vi "VIH HelpGen - Image - Find Ctrl Area in Conpane Picture - Preparation.vi"(9 "Ctrl Attributes":T2[](array[typedef]), 10 "Term Names":string[](array[string]), 11 "Ctrl Labels":string[](array[string])) -> (0 "Max Column - Indicators":i32, 1 "Max Column - Controls":i32, 3 "Params":T1(array[cluster]) {"Name image" format="%.0x"})   [LabVIEW 2014]
doc: "::: VI Helpeks :::\nCopyright (c) 2000-2026 Konstantin Shifershteyn. All rights reserved."
uses:
  VIH HelpGen Typedef - Control Terminal Attributes Cluster.ctl
panel:
  # "VI Helpeks\nCopyright (c) 2012-2026 Konstantin Shifershteyn"
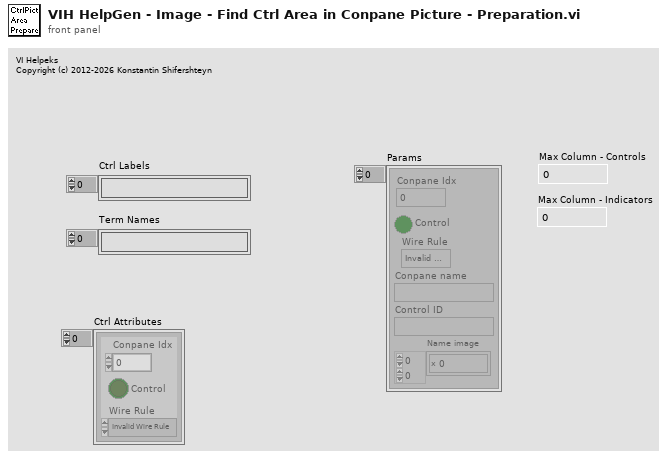
[diagram p1: front panel]
types:
  T1 = cluster{"Conpane Idx":i32, "Control":bool, "Wire Rule":enum16{"Invalid Wire Rule", "Required", "Recommended", "Optional", "Dynamic Dispatch"}, "Conpane name":string, "Control ID":string, "Name image":u32[][]}[]
  T2 = typedef "VIH HelpGen Typedef - Control Terminal Attributes Cluster.ctl" = cluster{"Conpane Idx":i32, "Control":bool, "Wire Rule":enum16{"Invalid Wire Rule", "Required", "Recommended", "Optional", "Dynamic Dispatch"}}
  T3 = cluster{i32, "Conpane name out":string, "Control ID":string, i32}
  T4 = cluster{i32, "Conpane name out":string, "Control ID":string, i32}[]
  T5 = enum16{"Invalid Wire Rule", "Required", "Recommended", "Optional", "Dynamic Dispatch"}
  T6 = cluster{"Conpane Idx":i32, "Control":bool, "Wire Rule":enum16{"Invalid Wire Rule", "Required", "Recommended", "Optional", "Dynamic Dispatch"}, "Conpane name out":string, "Control ID":string, "Image 2D Array":u32[][]}
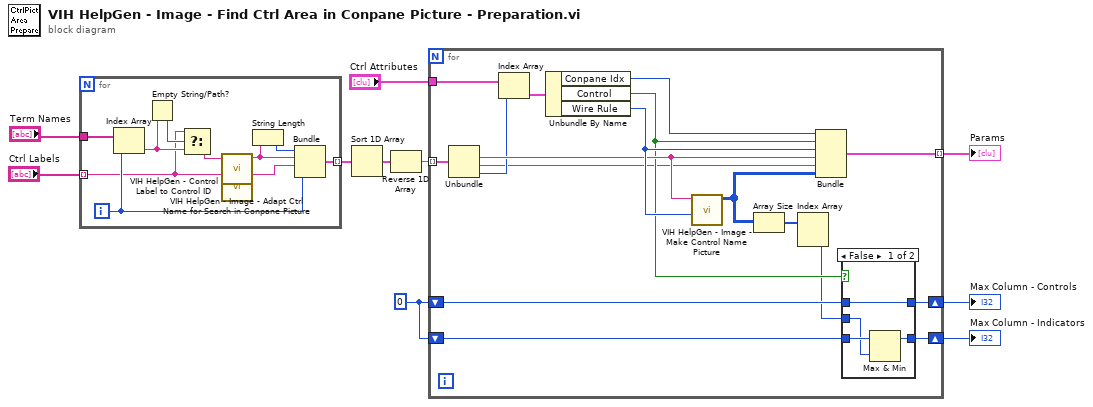
[diagram p0: block diagram]
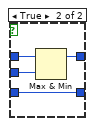
[diagram p2: hidden frame]
diagram:
  w4 = 0
  n1 = for {
    tunnel: [w19] -> w10 mode=indexing
    tunnel: "Ctrl Labels" -> [w12] mode=indexing
    tunnel: "Term Names" -> [w16]
    i -> [w15]
    n2 = Index Array(array=w16, index=w15) -> (element=w14:string)
    n3 = Empty String/Path?(string/path=w14) -> (empty?=w13:bool)
    n4 = Select(t=w12, s=w13, f=w14) -> (s? t:f=w11:string)
    n5 = call "VIH HelpGen - Image - Adapt Ctrl Name for Search in Conpane Picture.vi"("name"=w11) -> ("Conpane name out"=w18:string)  [unwired: 10 in]
    n6 = call "VIH HelpGen - Control Label to Control ID.vi"("Control Name"=w12) -> ("Control ID"=w17:string)  [unwired: 10 in]
    n7 = String Length(string=w18) -> (length=w20:i32)
    n8 = Bundle(w20, "Conpane name out"=w18, "Control ID"=w17, w15) -> (w19:T3)  [unwired: 1 in]
  }
  n9 = Sort 1D Array(array=w10) -> (sorted array=w8:T4)
  n10 = Reverse 1D Array(array=w8) -> (reversed array=w7:T4)
  n11 = for {
    tunnel: w7 -> [w37] mode=indexing
    tunnel: "Ctrl Attributes" -> [w36]
    tunnel: [w31] -> w5 mode=indexing
    shift-right: [w25] -> w3
    shift-left: w4 -> [w24]
    shift-right: [w27] -> w2
    shift-left: w4 -> [w26]
    n12 = Unbundle(w37) -> ("Conpane name out"=w32:string, "Control ID"=w21:string, w22:i32)  [unwired: 1 out]
    n13 = Index Array(array=w36, index=w22) -> (element=w35:T2)
    n14 = Unbundle By Name(w35) -> ("Conpane Idx"=w34:i32, "Control"=w28:bool, "Wire Rule"=w33:T5)
    n15 = call "VIH HelpGen - Image - Make Control Name Picture.vi"("Wire Rule"=w33, "Control name"=w32) -> ("Image 2D Array"=w30:u32[][])  [unwired: 9 in]
    n16 = Array Size(array=w30) -> (size(s)=w29:i32[])
    n17 = Index Array(array=w29) -> (element #2=w23:i32)  [unwired: 2 in, 1 out]
    n18 = Bundle("Conpane Idx"=w34, "Control"=w28, "Wire Rule"=w33, "Conpane name out"=w32, "Control ID"=w21, "Image 2D Array"=w30) -> (w31:T6)  [unwired: 1 in]
    n19 = case shown="False" w28 {
      tunnel: [w39 w45] -> w27
      tunnel: w26 -> [w40 w45]
      tunnel: [w41 w43] -> w25
      tunnel: w24 -> [w41 w44]
      tunnel: w23 -> [w38 w42]
      frame False {
        n20 = Max & Min(x=w40, y=w38) -> (max(x,y)=w39:i32)  [unwired: 1 out]
      }
      frame True {
        n21 = Max & Min(x=w44, y=w42) -> (max(x,y)=w43:i32)  [unwired: 1 out]
      }
    }
  }
  "Params" <- w5
  "Max Column - Controls" <- w3
  "Max Column - Indicators" <- w2
